vi "Find Background Image.vi"(10 "Backgroundic Qualities":T1(array[cluster]), 11 "Images":refnum<class "SVGImage.lvclass">[](array[class])) -> (2 "Backgroundic Qualities":T2, 3 "Background Image":refnum<class "SVGImage.lvclass">, 5 "Index":i32)   [LabVIEW 2019, in "SVGImage.lvclass"]
uses:
  SVGImage.lvclass
  C:/Users/Albro/Documents/GitHub/AFM-Lithography/lvsrc/Classes/Parse/SVG Object/SVG Object.lvclass
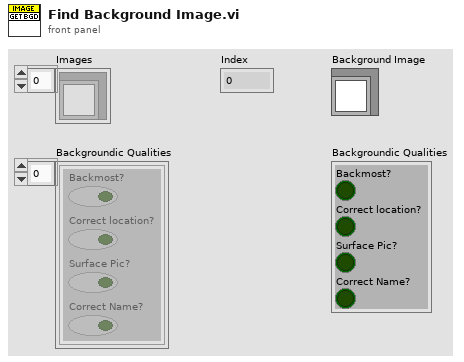
[diagram p1: front panel]
types:
  T1 = cluster{"Backmost?":bool, "Correct location?":bool, "Surface Pic?":bool, "Correct Name?":bool}[]
  T2 = cluster{"Backmost?":bool, "Correct location?":bool, "Surface Pic?":bool, "Correct Name?":bool}
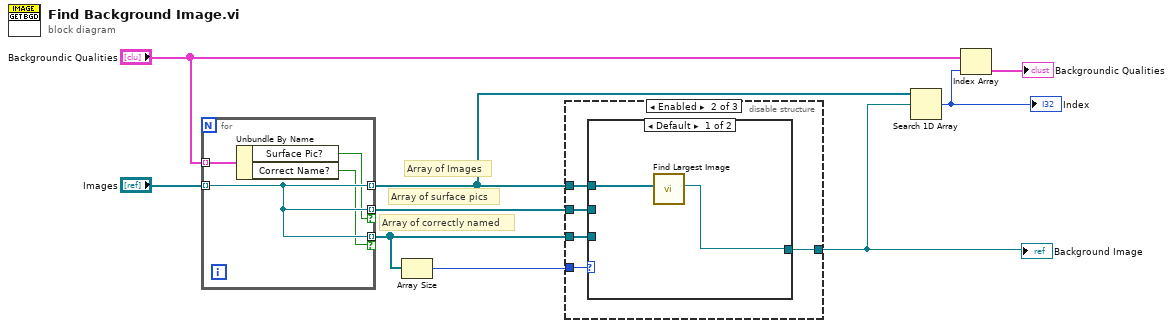
[diagram p0: block diagram]
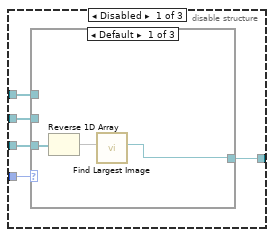
[diagram p2: hidden frame]
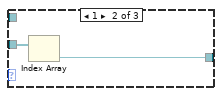
[diagram p3: hidden frame]
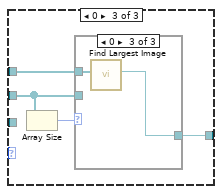
[diagram p4: hidden frame]
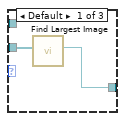
[diagram p5: hidden frame]
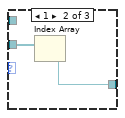
[diagram p6: hidden frame]
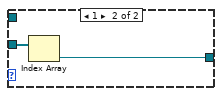
[diagram p7: hidden frame]
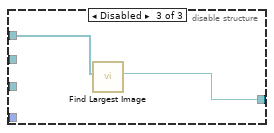
[diagram p8: hidden frame]
diagram:
  # "Array of correctly named"
  # "Array of surface pics"
  # "Array of Images"
  n1 = for {
    tunnel: "Backgroundic Qualities" -> [w13] mode=indexing
    tunnel: "Images" -> [w12] mode=indexing
    tunnel: [w12] -> w6 mode=indexing
    tunnel: [w12] -> w7 mode=indexing if=w10
    tunnel: [w12] -> w8 mode=indexing if=w11
    n2 = Unbundle By Name(w13) -> ("Surface Pic?"=w10:bool, "Correct Name?"=w11:bool)
  }
  n3 = Array Size(array=w8) -> (size(s)=w9:i32)
  n4 = disable-structure shown="Enabled" {
    disable-tunnel: w9 -> [w18 w38 _]
    disable-tunnel: w8 -> [w17 w37 _]
    disable-tunnel: w7 -> [w16 w36 _]
    disable-tunnel: w6 -> [w15 w35 w44]
    disable-tunnel: [w14 w34 w43] -> w5
    frame Disabled {
      n5 = case shown="Default" w18 {
        tunnel: w17 -> [w21 w23 _]
        tunnel: [w19 w22 w25] -> w14
        tunnel: w16 -> [_ _ w24]
        tunnel: w15 -> [_ _ w26]
        frame Default {
          n6 = Reverse 1D Array(array=w21) -> (reversed array=w20:refnum<class "SVGImage.lvclass">[])
          n7 = call "Find Largest Image.vi"("Images"=w20) -> ("Largest Image"=w19:refnum<class "SVGImage.lvclass">)  [unwired: 10 in]
        }
        frame 1 {
          n8 = Index Array(array=w23) -> (element=w22:refnum<class "SVGImage.lvclass">)  [unwired: 1 in]
        }
        frame 0 {
          n9 = Array Size(array=w24) -> (size(s)=w27:i32)
          n10 = case shown="0" w27 {
            tunnel: w26 -> [_ _ w33]
            tunnel: [w28 w30 w32] -> w25
            tunnel: w24 -> [w29 w31 _]
            frame Default {
              n11 = call "Find Largest Image.vi"("Images"=w29) -> ("Largest Image"=w28:refnum<class "SVGImage.lvclass">)  [unwired: 10 in]
            }
            frame 1 {
              n12 = Index Array(array=w31) -> (element=w30:refnum<class "SVGImage.lvclass">)  [unwired: 1 in]
            }
            frame 0 {
              n13 = call "Find Largest Image.vi"("Images"=w33) -> ("Largest Image"=w32:refnum<class "SVGImage.lvclass">)  [unwired: 10 in]
            }
          }
        }
      }
    }
    frame Enabled {
      n14 = case shown="Default" w38 {
        tunnel: w37 -> [_ w42]
        tunnel: [w40 w41] -> w34
        tunnel: w36 -> [_ _]
        tunnel: w35 -> [w39 _]
        frame Default {
          n15 = call "Find Largest Image.vi"("Images"=w39) -> ("Largest Image"=w40:refnum<class "SVGImage.lvclass">)  [unwired: 10 in]
        }
        frame 1 {
          n16 = Index Array(array=w42) -> (element=w41:refnum<class "SVGImage.lvclass">)  [unwired: 1 in]
        }
      }
    }
    frame Disabled {
      n17 = call "Find Largest Image.vi"("Images"=w44) -> ("Largest Image"=w43:refnum<class "SVGImage.lvclass">)  [unwired: 10 in]
    }
  }
  "Background Image" <- w5
  n18 = Search 1D Array(1D array=w6, element=w5) -> (index of element=w4:i32)  [unwired: 1 in]
  "Index" <- w4
  n19 = Index Array(array="Backgroundic Qualities", index=w4) -> (element=→"Backgroundic Qualities":T2)
